vi "Test_C_Helpers.vi"() -> ()   [LabVIEW 2021]
uses:
  CANsub_C.lvlib
  common/Typedefs/Bytes.ctl
  common/CANsub_Common.lvlib
  common/Typedefs/Payload.ctl
  codec_vis/CANsub_Codec.lvlib
  common/Typedefs/CAN_Frame.ctl
panel:
  out "ping payload":u8[](array[numeric]) format="%.0x"
  out "error out":errorcluster
  out "ping received":bool
  out "peer close":bool
  out "decode errors":i32
  out "crc errors":u32
  out "mismatches":u32
  out "frames received":i32
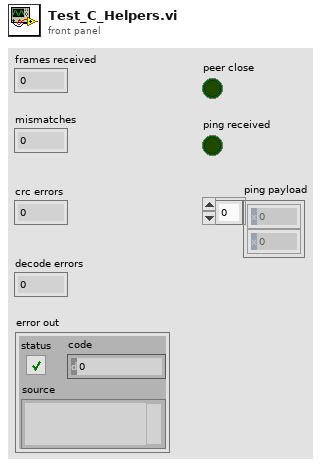
[diagram p1: front panel]
types:
  T1 = typedef "CANsub_Common.lvlib/CAN_Frame.ctl" = cluster{"t_dev":dbl, "id":u32, "ide":bool, "fdf":bool, "rtr":bool, "brs":bool, "esi":bool, "tx_ack":bool, "error":bool, "err type":u8, "dlc":u8, "data":T2}
  T2 = typedef "CANsub_Common.lvlib/Bytes.ctl" = u8[]
  T3 = typedef "CANsub_Common.lvlib/Payload.ctl" = cluster{"payload":T2}
  T4 = typedef "CANsub_C.lvlib/C_State.ctl" = u8[]
  T5 = typedef "CANsub_C.lvlib/C_Decode_Result.ctl" = cluster{"n frames":i32, "peer close":bool, "ping len":i32, "crc errors":u32, "decode errors":i32}
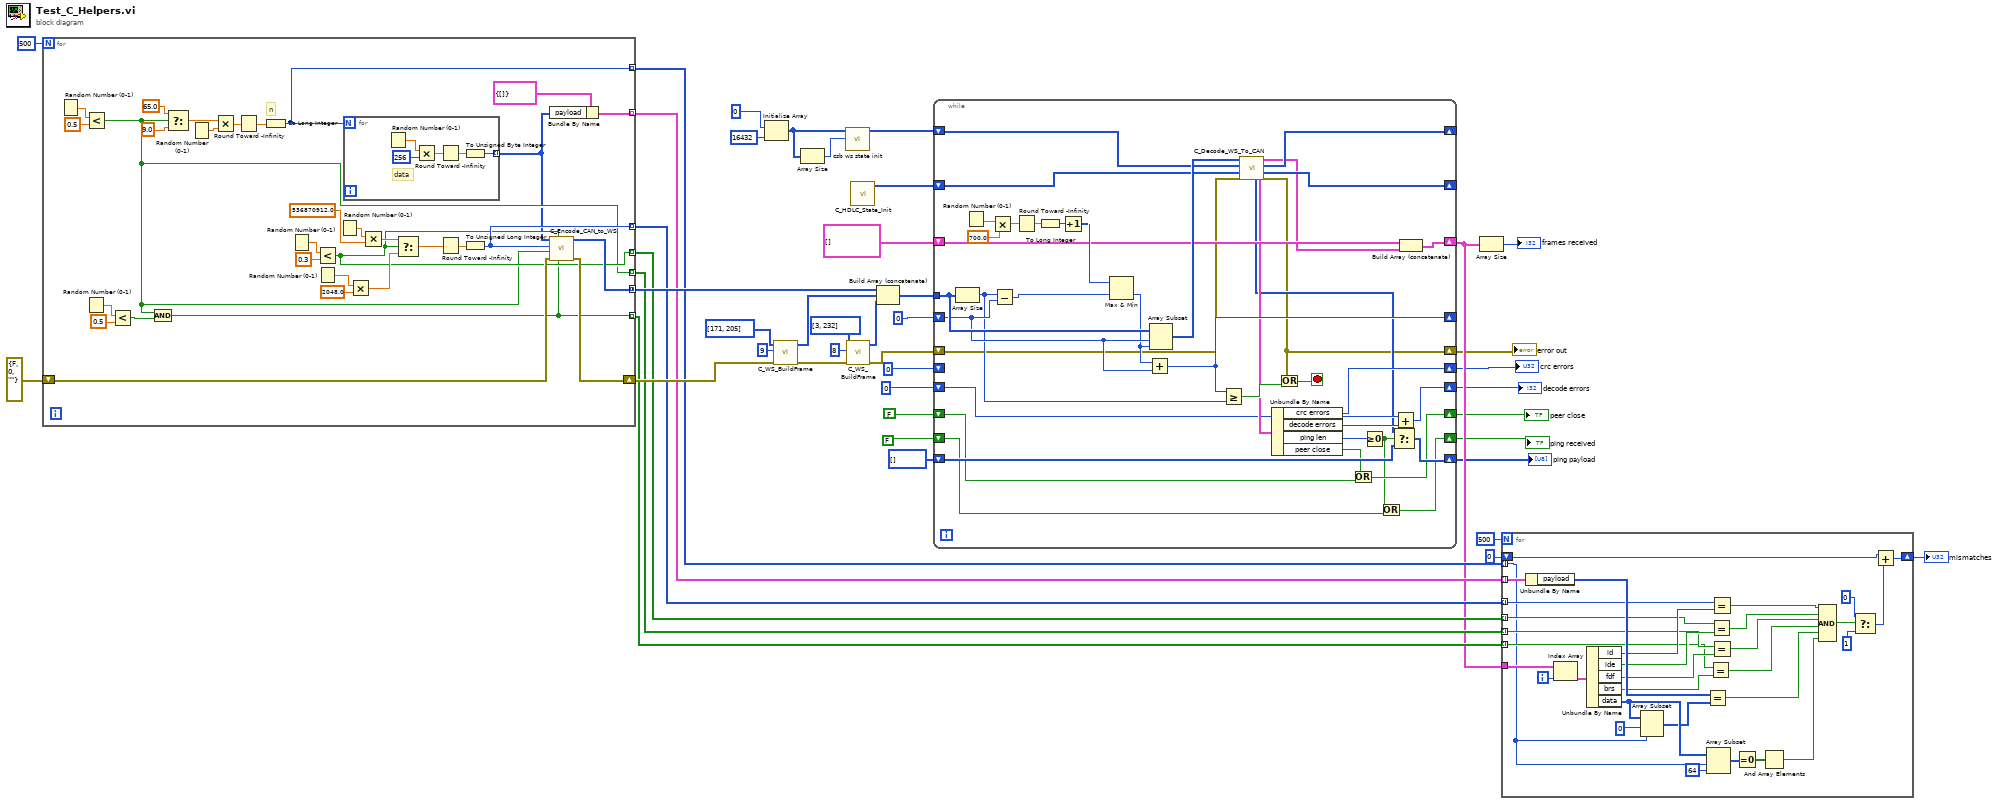
[diagram p0: block diagram]
diagram:
  n1 = for {
    N: 500 -> [_]
    shift-right: [w52] -> w40
    shift-left: errorcluster {"status"=FALSE, "code"=0, "source"=""} ("error constant") -> [w53]
    tunnel: [w54] -> w41 mode=concatenating
    tunnel: [w51] -> w14 mode=indexing
    tunnel: [w50] -> w13 mode=indexing
    tunnel: [w49] -> w11 mode=indexing
    tunnel: [w48] -> w12 mode=indexing
    tunnel: [w45] -> w15 mode=indexing
    tunnel: [w44] -> w16 mode=indexing
    # "n"
    n2 = Random Number (0-1)() -> (number: 0 to 1=w75:dbl)
    n3 = Less?(x=w75, y=0.5) -> (x < y?=w48:bool)
    n4 = Random Number (0-1)() -> (number: 0 to 1=w72:dbl)
    n5 = Less?(x=w72, y=0.5) -> (x < y?=w71:bool)
    n6 = And(x=w48, y=w71) -> (x .and. y?=w49:bool)
    n7 = Select(t=65.0, s=w48, f=9.0) -> (s? t:f=w58:dbl)
    n8 = Random Number (0-1)() -> (number: 0 to 1=w57:dbl)
    n9 = Multiply(x=w58, y=w57) -> (x*y=w56:dbl)
    n10 = Round Toward -Infinity(1:w56) -> (0:w55:dbl)
    n11 = To Long Integer(number=w55) -> (32bit integer=w44:i32)
    n12 = Random Number (0-1)() -> (number: 0 to 1=w69:dbl)
    n13 = Less?(x=w69, y=0.3) -> (x < y?=w50:bool)
    n14 = Random Number (0-1)() -> (number: 0 to 1=w65:dbl)
    n15 = Random Number (0-1)() -> (number: 0 to 1=w68:dbl)
    n16 = for {
      N: w44 -> [_]
      tunnel: [w76] -> w46 mode=indexing
      # "data"
      n17 = Random Number (0-1)() -> (number: 0 to 1=w80:dbl)
      n18 = Multiply(x=w80, y=256) -> (x*y=w78:dbl)
      n19 = Round Toward -Infinity(1:w78) -> (0:w77:dbl)
      n20 = To Unsigned Byte Integer(number=w77) -> (unsigned 8bit integer=w76:u8)
    }
    n21 = Multiply(x=w65, y=2048.0) -> (x*y=w63:dbl)
    n22 = Multiply(x=w68, y=536870912.0) -> (x*y=w64:dbl)
    n23 = Select(t=w64, s=w50, f=w63) -> (s? t:f=w62:dbl)
    n24 = Round Toward -Infinity(1:w62) -> (0:w61:dbl)
    n25 = To Unsigned Long Integer(number=w61) -> (unsigned 32bit integer=w51:u32)
    n26 = Bundle By Name(cluster=T3 {"payload"=[]} ("Payload"), "payload"=w46) -> (w45:T3)
    n27 = call "C_Encode_CAN_to_WS.vi"("brs"=w49, "ide"=w50, "error in (no error)"=w53, "fdf"=w48, "id"=w51, "data"=w46) -> ("error out"=w52:errorcluster, "ws frame"=w54:u8[])  [unwired: 4 in]
  }
  n28 = Initialize Array(u8 0, 16432 ("dimension size")) -> (w30:u8[])
  n29 = call "C_WS_BuildFrame.vi"("error in (no error)"=w40, "opcode"=u8 9, "payload"=u8[] [171, 205]) -> ("error out"=w39:errorcluster, "frame"=w38:u8[])  [unwired: 7 in]
  n30 = Array Size(array=w30) -> (size(s)=w29:i32)
  n31 = call "csb ws state init.vi"("state_size"=w29, "state"=w30) -> ("state_out"=w28:u8[])  [unwired: 7 in, 2 out]
  n32 = call "C_WS_BuildFrame.vi"("error in (no error)"=w39, "opcode"=u8 8, "payload"=u8[] [3, 232]) -> ("error out"=w20:errorcluster, "frame"=w37:u8[])  [unwired: 7 in]
  n33 = call "C_HDLC_State_Init.vi"() -> ("C_State"=w27:T4)  [unwired: 10 in, 1 out]
  n34 = Build Array (concatenate)(w41, w38, w37) -> (w19:u8[])
  n35 = while {
    shift-right: [w105] -> _
    shift-left: w28 -> [w108]
    shift-right: [w106] -> _
    shift-left: w27 -> [w107]
    shift-right: [w104] -> _
    shift-left: 0 -> [w111]
    shift-right: [w98] -> w8
    shift-left: T1[] [] -> [w100]
    shift-right: [w84] -> w4
    shift-left: FALSE -> [w85]
    shift-right: [w81] -> w5
    shift-left: FALSE -> [w82]
    shift-right: [w96] -> w3
    shift-left: u32 0 -> [_]
    shift-right: [w93] -> w2
    shift-left: 0 -> [w94]
    shift-right: [w87] -> w6
    shift-left: w20 -> [w88]
    tunnel: w19 -> [w112]
    shift-right: [w90] -> w1
    shift-left: u8[] [] ("ping payload") -> [w89]
    stop <- w102 stop-if-true
    n36 = Array Size(array=w112) -> (size(s)=w101:i32)
    n37 = Random Number (0-1)() -> (number: 0 to 1=w119:dbl)
    n38 = Multiply(x=w119, y=700.0) -> (x*y=w117:dbl)
    n39 = Subtract(x=w101, y=w111) -> (x-y=w114:i32)
    n40 = Round Toward -Infinity(1:w117) -> (0:w116:dbl)
    n41 = To Long Integer(number=w116) -> (32bit integer=w115:i32)
    n42 = Increment(x=w115) -> (x+1=w113:i32)
    n43 = Max & Min(x=w113, y=w114) -> (min(x,y)=w110:i32)  [unwired: 1 out]
    n44 = Add(x=w110, y=w111) -> (x+y=w104:i32)
    n45 = Array Subset(array=w112, index=w111, length=w110) -> (w109:u8[])
    n46 = Greater Or Equal?(x=w104, y=w101) -> (x >= y?=w103:bool)
    n47 = call "C_Decode_WS_To_CAN.vi"("error in (no error)"=w88, "hdlc state in"=w107, "ws state in"=w108, "bytes in"=w109) -> ("error out"=w87:errorcluster, "hdlc state out"=w106:T4, "ws state out"=w105:T4, "frames"=w99:T1[], "ping payload"=w91:u8[], "result"=w97:T5)  [unwired: 2 in]
    n48 = Unbundle By Name(w97) -> ("crc errors"=w96:u32, "decode errors"=w95:i32, "ping len"=w92:i32, "peer close"=w86:bool)
    n49 = Or(x=w87, y=w103) -> (x .or. y?=w102:bool)
    n50 = Or(x=w86, y=w85) -> (x .or. y?=w84:bool)
    n51 = Greater Or Equal To 0?(x=w92) -> (x >= 0?=w83:bool)
    n52 = Or(x=w83, y=w82) -> (x .or. y?=w81:bool)
    n53 = Select(t=w91, s=w83, f=w89) -> (s? t:f=w90:u8[])
    n54 = Add(x=w94, y=w95) -> (x+y=w93:i32)
    n55 = Build Array (concatenate)(w100, w99) -> (w98:T1[])
  }
  "crc errors" <- w3
  "decode errors" <- w2
  "peer close" <- w4
  "ping received" <- w5
  "error out" <- w6
  "ping payload" <- w1
  n56 = Array Size(array=w8) -> (size(s)=→"frames received":i32)
  n57 = for {
    N: 500 -> [_]
    tunnel: w16 -> [w121] mode=indexing
    tunnel: w15 -> [w148] mode=indexing
    tunnel: w14 -> [w146] mode=indexing
    tunnel: w13 -> [w144] mode=indexing
    tunnel: w12 -> [w142] mode=indexing
    tunnel: w11 -> [w140] mode=indexing
    tunnel: w8 -> [w151]
    shift-right: [w125] -> w9
    shift-left: 0 -> [w124]
    i -> [w150]
    n58 = Unbundle By Name(w148) -> ("payload"=w147:T2)
    n59 = Index Array(array=w151, index=w150) -> (element=w149:T1)
    n60 = Unbundle By Name(w149) -> ("id"=w145:u32, "ide"=w143:bool, "fdf"=w141:bool, "brs"=w139:bool, "data"=w123:T2)
    n61 = Array Subset(array=w123, index=0, length=w121) -> (w120:T2)
    n62 = Equal?(x=w147, y=w120) -> (x = y?=w134:bool)
    n63 = Array Subset(array=w123, index=w121, length=64) -> (w137:T2)
    n64 = Equal?(x=w140, y=w139) -> (x = y?=w133:bool)
    n65 = Equal?(x=w144, y=w143) -> (x = y?=w131:bool)
    n66 = Equal?(x=w146, y=w145) -> (x = y?=w130:bool)
    n67 = Equal?(x=w142, y=w141) -> (x = y?=w132:bool)
    n68 = Equal To 0?(x=w137) -> (x = 0?=w136:bool[])
    n69 = And Array Elements(Boolean array=w136) -> (logical AND=w135:bool)
    n70 = Compound Arithmetic op=AND(w130, w131, w132, w133, w134, w135) -> (w129:bool)
    n71 = Select(t=0, s=w129, f=1) -> (s? t:f=w126:i32)
    n72 = Add(x=w124, y=w126) -> (x+y=w125:i32)
  }
  "mismatches" <- w9
